vi "libssh2_knownhost_free.vi"(8 "error in (no error)":errorcluster, 11 "host key database":T1) -> (0 "error out":errorcluster)   [LabVIEW 2017, in "libssh2.lvlib"]
doc: "Release memory associated with a host key database."
uses:
  libssh2.lvlib
  Host Key Database Refnum.ctl
  Global Settings.vi
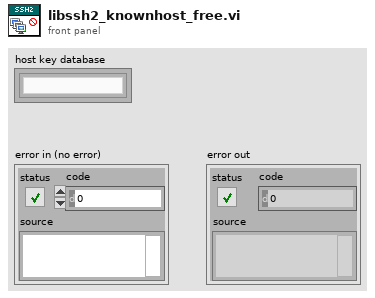
[diagram p1: front panel]
types:
  T1 = typedef "libssh2.lvlib/Host Key Database Refnum.ctl" = refnum<k1>
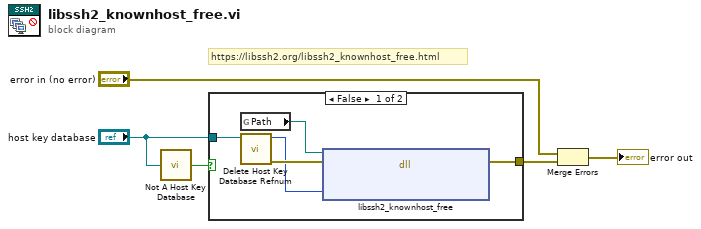
[diagram p0: block diagram]
diagram:
  # "https://libssh2.org/libssh2_knownhost_free.html"
  n1 = call "Not A Host Key Database.vi"("host key database"="host key database") -> ("Not a Host Key Database?"=w1:bool)
  n2 = case shown="False" w1 {
    tunnel: [w10 _] -> w5
    tunnel: "host key database" -> [w8 _]
    frame False {
      n3 = global read "Global Settings.vi" "Path"() -> (w6:path)
      n4 = call "Delete Host Key Database Refnum.vi"("host key database"=w8) -> ("error out"=w9:errorcluster, "LIBSSH2_KNOWNHOSTS*"=w7:u64)  [unwired: 9 in]
      n5 = dll-call lib="?" fn="libssh2_knownhost_free"(path in=w6, error in=w9, "hosts"=w7) -> (error out=w10:errorcluster)  [unwired: 3 in, 1 out]
    }
    frame True {
    }
  }
  n6 = Merge Errors("error in (no error)", w5) -> (→"error out":errorcluster)
